vi "create default channels.vi"() -> (0 "error out":errorcluster, 2 "channels":refnum<class "TBM channel.lvclass">[](array[class]), 3 "module":refnum<class "tag select module configuration.lvclass">, 5 "instance identifier":string)   [LabVIEW 2015, in "tag select module tests.lvlib"]
uses:
  tag select module tests.lvlib
  <vilib>/NI/Tag Bus Module Framework/channel/TBM channel.lvclass
  module/configuration/tag select module configuration.lvclass
  <vilib>/NI/Tag Bus/tag/Data Type.ctl
  <vilib>/NI/Configuration Framework/serializable configuration/NISE_CEF_serializable configuration.lvclass
  <vilib>/NI/Tag Bus/tag/tag descriptor.lvclass
panel:
  in  "Data Type":T1
  out "Array":string[](array[string])
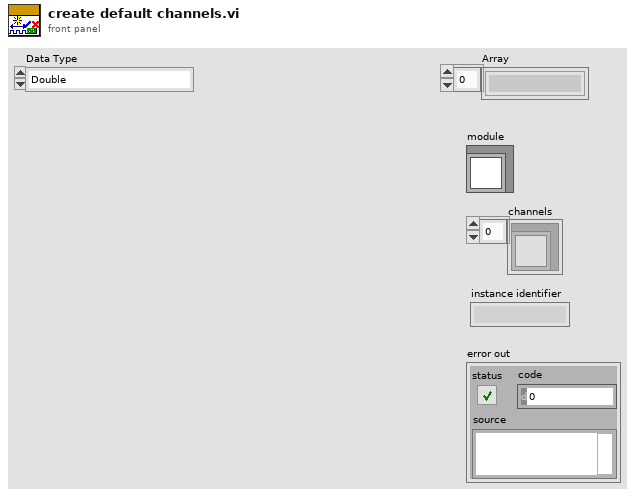
[diagram p1: front panel]
types:
  T1 = typedef "tag bus.lvlib/tag descriptor.lvclass/Data Type.ctl" = enum16{"Double", "Single", "I64", "I32", "I16", "I8", "U64", "U32", "U16", "U8", "Boolean", "String", "Array of Double", "Array of Single", "Array of I64", "Array of I32", "Array of I16", "Array of I8", "Array of U64", "Array of U32", "Array of U16", "Array of U8", "Array of Boolean", "Array of String"}
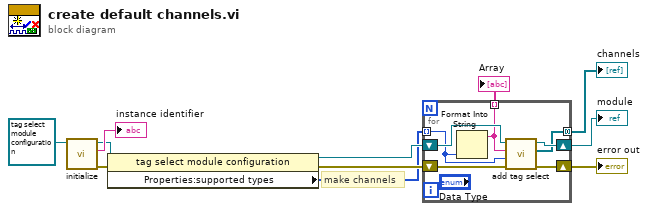
[diagram p0: block diagram]
diagram:
  # "make channels"
  n1 = call <vilib>:"initialize.vi"("configuration in"=refnum<class "tag select module configuration.lvclass"> refnum ("tag bus configurable plugin module configuration")) -> ("error out"=w9:errorcluster, "identifier"=→"instance identifier":string, "configuration out"=w7:refnum<class "tag select module configuration.lvclass">)  [unwired: 8 in]
  n2 = property class="tag select module configuration"(reference=w7, error in=w9) -> (reference out=w4:refnum<class "tag select module configuration.lvclass">, error out=w8:errorcluster, "Properties:supported types"=w2:T1[])
  n3 = for {
    shift-right: [w17] -> w6
    shift-left: w4 -> [w18]
    shift-right: [w16] -> w11
    shift-left: w8 -> [w14]
    tunnel: [w15] -> w3 mode=concatenating
    tunnel: w2 -> [w13] mode=indexing
    tunnel: [w12] -> w1 mode=indexing
    n4 = Format Into String(w13) -> (resulting string=w12:string)  [unwired: 3 in, 1 out]
    n5 = call "add tag select.vi"("error in"=w14, "data type"=w13, "tag select name"=w12, "tag select module configuration in"=w18) -> ("error out"=w16:errorcluster, "created channels"=w15:refnum<class "TBM channel.lvclass">[], "tag select module configuration out"=w17:refnum<class "tag select module configuration.lvclass">)  [unwired: 5 in]
  }
  "error out" <- w11
  "channels" <- w3
  "module" <- w6
  "Array" <- w1
